vi "test invalid input response.vi"(8 "error in (no error)":errorcluster) -> (0 "error out":errorcluster, 3 "body":string)   [LabVIEW 2020, in "MCP Server tests.lvlib"]
doc: "Test 76: an inputResponses entry that is not a valid answer is asked again.\n\nMCP 2026-07-28 says a server should validate inputResponses and re-request missing or invalid input. Ask User.vi (through Confirm With User.vi in the fixture fake_tool_confirm, key confirm_action) treats an entry that is not a JSON object with action accept, decline or cancel as not answered (Valid Input Response.vi). Before, such an entry counted as cancel and the call completed.\n\n1. Modern tools/call with inputResponses {\"confirm_action\":42} -> resultType input_required with inputRequests.confirm_action again.\n2. With {\"confirm_action\":{\"action\":\"maybe\"}} -> input_required again.\n3. With {\"confirm_action\":{\"action\":\"accept\"}} -> a complete result with outcome confirmed (regression)."
uses:
  MCP Server tests.lvlib
  <vilib>/addons/_JKI Toolkits/Caraya/classes/Test/Test.lvclass
  <vilib>/addons/_JKI Toolkits/Caraya/classes/Assert/Assert.lvclass
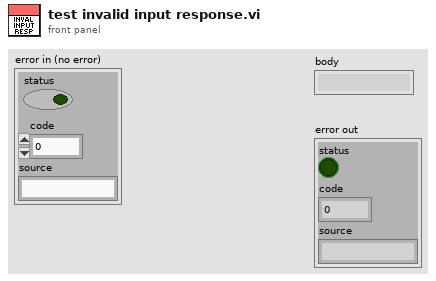
[diagram p1: front panel]
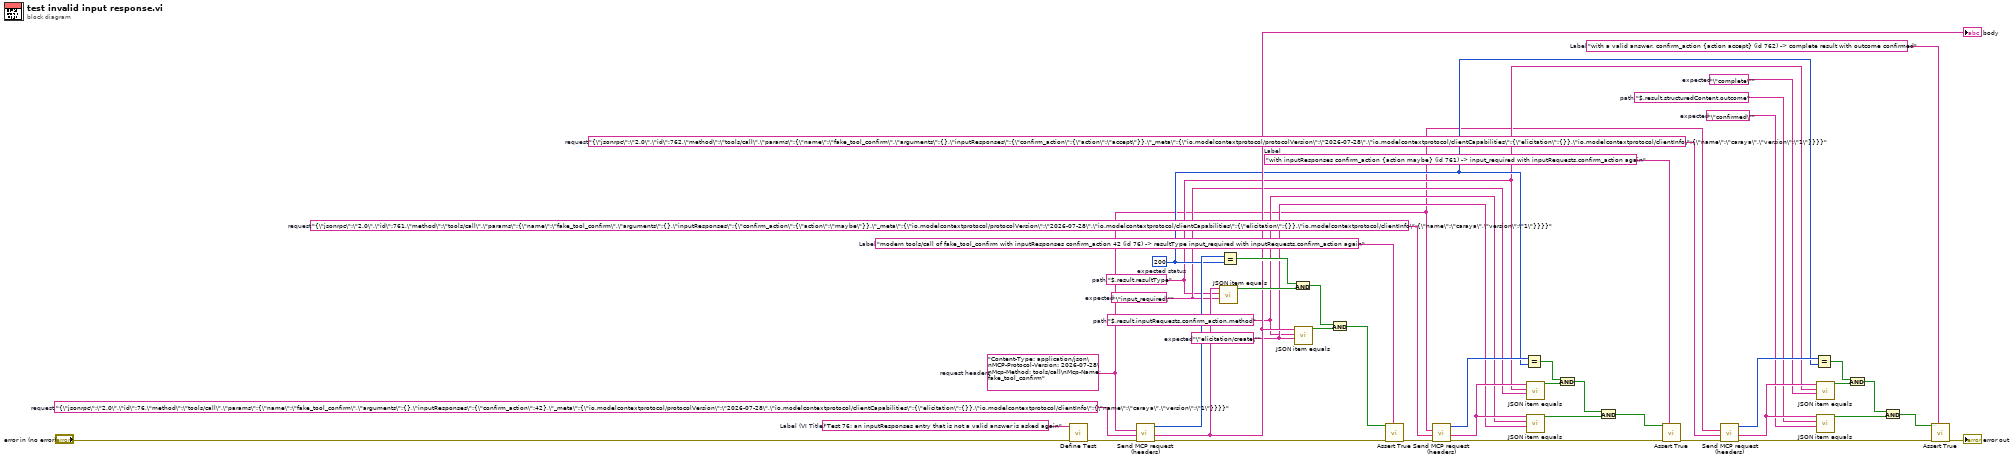
[diagram p0: block diagram]
diagram:
  w44 = "with a valid answer, confirm_action {action accept} (id 762) -> complete result with outcome confirmed"  # Label
  w34 = "with inputResponses confirm_action {action maybe} (id 761) -> input_required with inputRequests.confirm_action again"  # Label
  w24 = "modern tools/call of fake_tool_confirm with inputResponses confirm_action 42 (id 76) -> resultType input_required with inputRequests.confirm_action again"  # Label
  w15 = 200  # expected status
  w14 = "\"confirmed\""  # expected
  w13 = "$.result.structuredContent.outcome"  # path
  w12 = "\"complete\""  # expected
  w11 = "\"elicitation/create\""  # expected
  w10 = "$.result.inputRequests.confirm_action.method"  # path
  w9 = "\"input_required\""  # expected
  w8 = "$.result.resultType"  # path
  w7 = "{\"jsonrpc\":\"2.0\",\"id\":762,\"method\":\"tools/call\",\"params\":{\"name\":\"fake_tool_confirm\",\"arguments\":{},\"inputResponses\":{\"confirm_action\":{\"action\":\"accept\"}},\"_meta\":{\"io.modelcontextprotocol/protocolVersion\":\"2026-07-28\",\"io.modelcontextprotocol/clientCapabilities\":{\"elicitation\":{}},\"io.modelcontextprotocol/clientInfo\":{\"name\":\"caraya\",\"version\":\"1\"}}}}"  # request
  w6 = "{\"jsonrpc\":\"2.0\",\"id\":761,\"method\":\"tools/call\",\"params\":{\"name\":\"fake_tool_confirm\",\"arguments\":{},\"inputResponses\":{\"confirm_action\":{\"action\":\"maybe\"}},\"_meta\":{\"io.modelcontextprotocol/protocolVersion\":\"2026-07-28\",\"io.modelcontextprotocol/clientCapabilities\":{\"elicitation\":{}},\"io.modelcontextprotocol/clientInfo\":{\"name\":\"caraya\",\"version\":\"1\"}}}}"  # request
  w5 = "{\"jsonrpc\":\"2.0\",\"id\":76,\"method\":\"tools/call\",\"params\":{\"name\":\"fake_tool_confirm\",\"arguments\":{},\"inputResponses\":{\"confirm_action\":42},\"_meta\":{\"io.modelcontextprotocol/protocolVersion\":\"2026-07-28\",\"io.modelcontextprotocol/clientCapabilities\":{\"elicitation\":{}},\"io.modelcontextprotocol/clientInfo\":{\"name\":\"caraya\",\"version\":\"1\"}}}}"  # request
  w4 = "Content-Type: application/json\nMCP-Protocol-Version: 2026-07-28\nMcp-Method: tools/call\nMcp-Name: fake_tool_confirm"  # request headers
  w2 = "Test 76: an inputResponses entry that is not a valid answer is asked again"  # Label (VI Title)
  n1 = call <vilib>:"Define Test.vi"("error in (no error)"="error in (no error)", "Label (VI Title)"=w2) -> ("error out"=w3:errorcluster)  [unwired: 8 in, 1 out]
  n2 = call "Send MCP request (headers).vi"("error in (no error)"=w3, "request"=w5, "request headers"=w4) -> ("error out"=w16:errorcluster, "response"=w17:string, "status code"=w18:i32)  [unwired: 5 in, 1 out]
  "body" <- w17
  n3 = call "JSON item equals.vi"("expected"=w9, "path"=w8, "JSON"=w17) -> ("equal?"=w20:bool)  [unwired: 6 in, 2 out]
  n4 = Equal?(x=w18, y=w15) -> (x = y?=w19:bool)
  n5 = And(x=w19, y=w20) -> (x .and. y?=w22:bool)
  n6 = call "JSON item equals.vi"("expected"=w11, "path"=w10, "JSON"=w17) -> ("equal?"=w21:bool)  [unwired: 6 in, 2 out]
  n7 = And(x=w22, y=w21) -> (x .and. y?=w23:bool)
  n8 = call <vilib>:"Assert True.vi"("Label"=w24, "error in (no error)"=w16, "True?"=w23) -> ("error out"=w25:errorcluster)  [unwired: 7 in, 1 out]
  n9 = call "Send MCP request (headers).vi"("error in (no error)"=w25, "request"=w6, "request headers"=w4) -> ("error out"=w26:errorcluster, "response"=w27:string, "status code"=w28:i32)  [unwired: 5 in, 1 out]
  n10 = Equal?(x=w28, y=w15) -> (x = y?=w29:bool)
  n11 = call "JSON item equals.vi"("expected"=w9, "path"=w8, "JSON"=w27) -> ("equal?"=w30:bool)  [unwired: 6 in, 2 out]
  n12 = call "JSON item equals.vi"("expected"=w11, "path"=w10, "JSON"=w27) -> ("equal?"=w31:bool)  [unwired: 6 in, 2 out]
  n13 = And(x=w29, y=w30) -> (x .and. y?=w32:bool)
  n14 = And(x=w32, y=w31) -> (x .and. y?=w33:bool)
  n15 = call <vilib>:"Assert True.vi"("Label"=w34, "error in (no error)"=w26, "True?"=w33) -> ("error out"=w35:errorcluster)  [unwired: 7 in, 1 out]
  n16 = call "Send MCP request (headers).vi"("error in (no error)"=w35, "request"=w7, "request headers"=w4) -> ("error out"=w36:errorcluster, "response"=w37:string, "status code"=w38:i32)  [unwired: 5 in, 1 out]
  n17 = Equal?(x=w38, y=w15) -> (x = y?=w39:bool)
  n18 = call "JSON item equals.vi"("expected"=w12, "path"=w8, "JSON"=w37) -> ("equal?"=w40:bool)  [unwired: 6 in, 2 out]
  n19 = call "JSON item equals.vi"("expected"=w14, "path"=w13, "JSON"=w37) -> ("equal?"=w41:bool)  [unwired: 6 in, 2 out]
  n20 = And(x=w39, y=w40) -> (x .and. y?=w42:bool)
  n21 = And(x=w42, y=w41) -> (x .and. y?=w43:bool)
  n22 = call <vilib>:"Assert True.vi"("Label"=w44, "error in (no error)"=w36, "True?"=w43) -> ("error out"=→"error out":errorcluster)  [unwired: 7 in, 1 out]
